vi "PicoScope3000aExampleRapidBlockBulk.vi"() -> ()   [LabVIEW 2009]
panel:
  in  "PS3207A/B device\non non-USB 3.0 Port":bool
  in  "PS34XXA/B\nUSB Powered":bool
  in  "Trigger Settings":T1 {"Trigger Direction" items=["Rising", "Falling"]}
  in  "Channel A Settings":T2 {"Range" items=["10 mV", "20 mV", "50 mV", "100 mV", "200 mV", "500 mV", "1 V", "2 V", "5 V", "10 V", "20 V", "50 V ", "100 V"]; "Coupling" items=["AC", "DC"]}
  in  "Rapid Block Acquisition Settings":T3
  out "Capture Complete":bool
  in  "Run":bool
  out "Channel A":i16[](graph)
  in  "Capture Index":i16 min=0
  in  "stop":bool
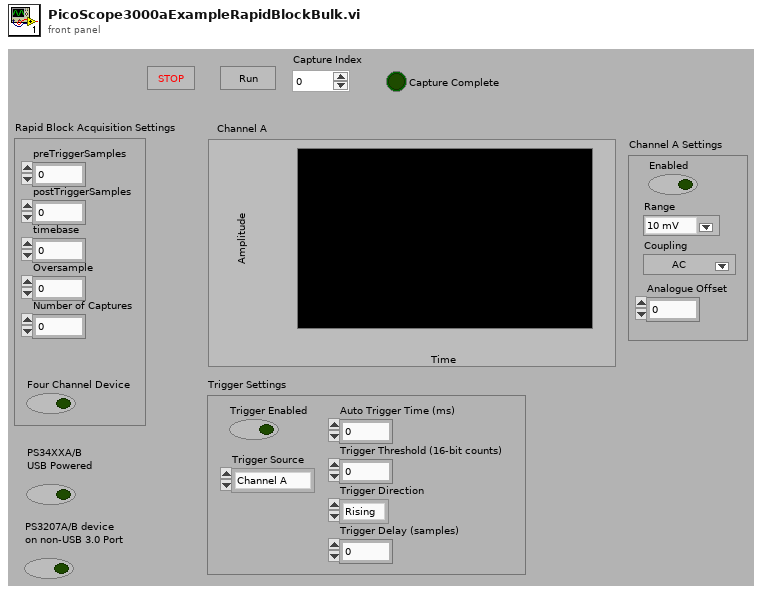
[diagram p1: front panel]
types:
  T1 = cluster{"Trigger Enabled":bool, "Trigger Source":enum16{"Channel A", "Channel B", "Channel C", "Channel D", "Ext."}, "Trigger Threshold (16-bit counts)":i16, "Trigger Direction":u16, "Trigger Delay (samples)":u32, "Auto Trigger Time (ms)":i16}
  T2 = cluster{"Enabled":bool, "Coupling":i16, "Range":u16, "Analogue Offset":sgl}
  T3 = cluster{"preTriggerSamples":u32, "postTriggerSamples":u32, "timebase":u32, "Four Channel Device":bool, "Oversample":i16, "Number of Captures":u32}
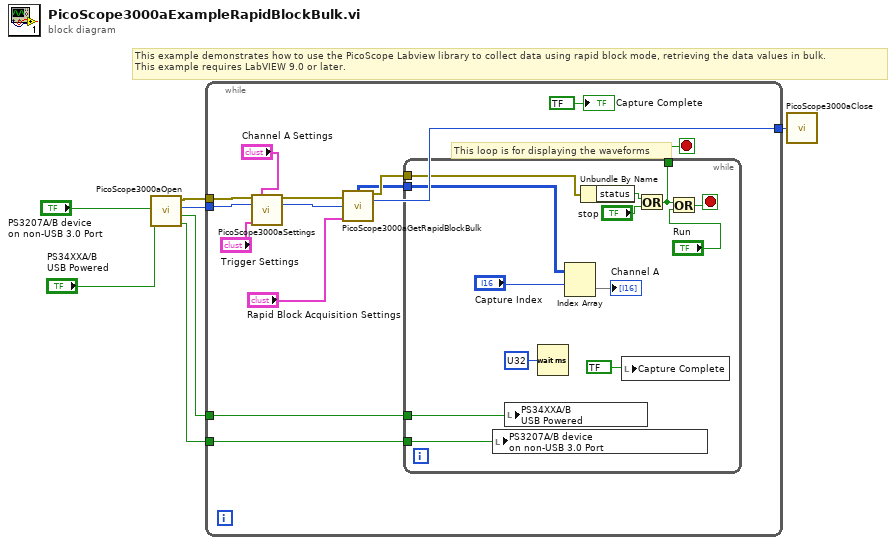
[diagram p0: block diagram]
diagram:
  # "This example demonstrates how to use the PicoScope Labview library to collect data using rapid block mode, retrieving the data values in bulk.\nThis example requires LabVIEW 9.0 or later."
  n1 = call "PicoScope3000aOpen.vi"("4-channel USB Powered"="PS34XXA/B\nUSB Powered", "2-channel USB 3.0 device on non-USB 3.0 Port"="PS3207A/B device\non non-USB 3.0 Port") -> ("2-channel USB 3.0 device on non-USB 3.0 Port Indication"=w1:bool, "4-channel USB Powered Indication"=w3:bool, "handle"=w5:i16, "error out"=w6:errorcluster)  [unwired: 4 in, 2 out]
  n2 = while {
    tunnel: [w16] -> w7
    tunnel: w6 -> [w11]
    tunnel: w5 -> [w10]
    tunnel: w3 -> [w9]
    tunnel: w1 -> [w8]
    stop <- w21 stop-if-true
    # "This loop is for displaying the waveforms"
    n3 = call "PicoScope3000aSettings.vi"("error in"=w11, "Channel A Settings"="Channel A Settings", "handle in"=w10, "Trigger Settings"="Trigger Settings") -> ("error out"=w14:errorcluster, "handle out"=w15:i16)  [unwired: 9 in, 1 out]
    n4 = call "PicoScope3000aGetRapidBlockBulk.vi"("error in"=w14, "handle in"=w15, "Rapid Block Acquisition Settings"="Rapid Block Acquisition Settings") -> ("Channel A Buffer"=w17:i16[][], "error out"=w18:errorcluster, "handle out"=w16:i16)  [unwired: 4 in, 6 out]
    n5 = while {
      tunnel: [w33] -> w21
      tunnel: w17 -> [w24]
      tunnel: w18 -> [w28]
      tunnel: w9 -> [w26]
      tunnel: w8 -> [w25]
      stop <- w32 stop-if-true
      n6 = local write "PS3207A/B device\non non-USB 3.0 Port"(w25) -> ()
      n7 = local write "PS34XXA/B\nUSB Powered"(w26) -> ()
      n8 = Wait (ms)(milliseconds to wait=u32 ?) -> ()  [unwired: 1 out]
      n9 = Index Array(array=w24, index (row)="Capture Index") -> (element=→"Channel A":i16[])  [unwired: 1 in]
      n10 = Unbundle By Name(w28) -> ("status"=w27:bool)
      n11 = local write "Capture Complete"(bool ? ("Capture Complete")) -> ()
      n12 = Or(x=w27, y="stop") -> (x .or. y?=w33:bool)
      n13 = Or(x=w33, y="Run") -> (x .or. y?=w32:bool)
    }
    "Capture Complete" <- bool ? ("Capture Complete")
  }
  n14 = call "PicoScope3000aClose.vi"("handle"=w7) -> ()
